vi "[ce] Get Win Module Path.vi"(8 "error in":errorcluster, 11 "Module Handle":u64 format="%.0x") -> (0 "error out":errorcluster, 2 "Path":path, 3 "dup Module Handle":u64 format="%.0x")   [LabVIEW 2021]
doc: "::: CalcExpress Toolkit :::\nCopyright (c) 2000-2026 Konstantin Shifershteyn. All rights reserved."
uses:
  kernel32.dll
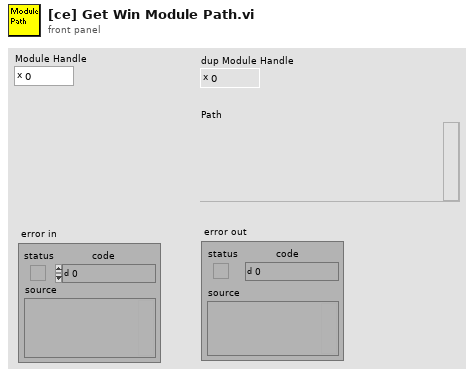
[diagram p1: front panel]
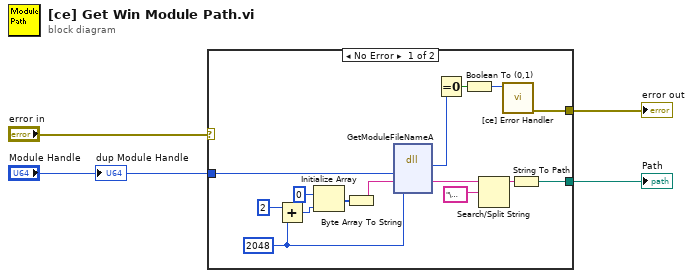
[diagram p0: block diagram]
diagram:
  n1 = case shown="No Error" "error in" {
    selector: "error in" -> [_ w20]
    tunnel: "Module Handle" -> [w19 _]
    tunnel: [w9 _] -> w4
    tunnel: [w5 w20] -> w2
    frame No Error {
      w13 = 2048 ("dimension size")
      n2 = Add(x=2 ("y"), y=w13) -> (x+y=w17:i32)
      n3 = Initialize Array(u8 0, w17) -> (w16:u8[])
      n4 = Byte Array To String(unsigned byte array=w16) -> (string=w15:string)
      n5 = dll-call lib="kernel32.dll" fn="GetModuleFileNameA"("HMODULE"=w19, "StrPnt"=w15, "StrLen"=w13) -> ("return type"=w8:i32, "StrPnt"=w12:string)  [unwired: 5 in, 2 out]
      n6 = Equal To 0?(x=w8) -> (x = 0?=w7:bool)
      n7 = Boolean To (0,1)(Boolean=w7) -> (0, 1=w6:i16)
      n8 = Search/Split String(string=w12, search string/char (-)="\u0000") -> (substring before match=w10:string)  [unwired: 1 in, 2 out]
      n9 = call "[ce] Error Handler.vi"("error code"=w6) -> ("error out"=w5:errorcluster)  [unwired: 9 in, 1 out]
      n10 = String To Path(string=w10) -> (path=w9:path)
    }
    frame Error {
    }
  }
  "Path" <- w4
  "error out" <- w2
  "dup Module Handle" <- "Module Handle"
